vi "Pascal's Triangle.vi"() -> ()   [LabVIEW 2026]
panel:
  out "Pascal's Triangle":dbl[][](array[numeric])
  in  "Number of Rows":i64
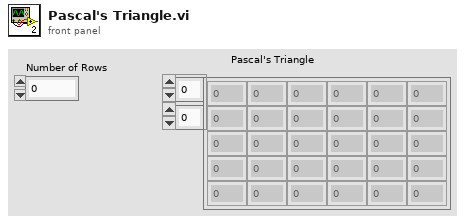
[diagram p1: front panel]
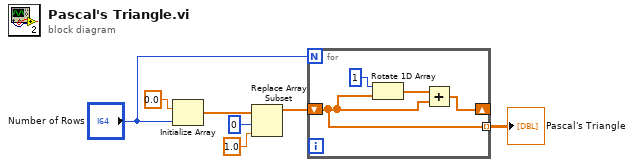
[diagram p0: block diagram]
diagram:
  n1 = Initialize Array(0.0 ("element"), "Number of Rows") -> (w5:dbl[])
  n2 = Replace Array Subset(array=w5, new element=1.0 ("new element/subarray"), index=0) -> (w2:dbl[])
  n3 = for {
    N: "Number of Rows" -> [_]
    shift-right: [w9] -> _
    shift-left: w2 -> [w8]
    tunnel: [w8] -> w1 mode=indexing
    n4 = Rotate 1D Array(1:w8, 2:1 ("n")) -> (0:w10:dbl[])
    n5 = Add(x=w10, y=w8) -> (x+y=w9:dbl[])
  }
  "Pascal's Triangle" <- w1
